vi "Read prelaunchSettings.vi"(8 "error in (no error)":errorcluster, 11 "ZM-ROOT-root in":refnum<class "ZM-ROOT-root.lvclass">) -> (0 "error out":errorcluster, 2 "ZM-ROOT-PRELAUNCH_SETTINGS":T1, 3 "ZM-ROOT-root out":refnum<class "ZM-ROOT-root.lvclass">)   [LabVIEW 2020, in "ZM-ROOT-root.lvlib" / "ZM-ROOT-root.lvclass"]
doc: "Reads one field of this class's private data. Generated by lvai_create_accessors from the class private data control."
uses:
  ZM-ROOT-root.lvclass
  ZM-ROOT-root.lvclass/ZM-ROOT-root.ctl
  ZM-ROOT-PRELAUNCH_SETTINGS.ctl
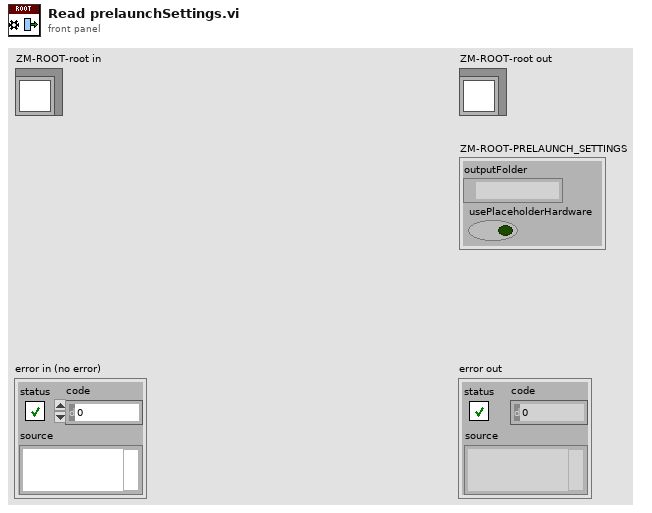
[diagram p1: front panel]
types:
  T1 = typedef "ZM-ROOT-root.lvlib/ZM-ROOT-root.lvclass/ZM-ROOT-PRELAUNCH_SETTINGS.ctl" = cluster{"outputFolder":path, "usePlaceholderHardware":bool}
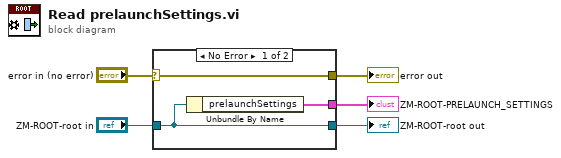
[diagram p0: block diagram]
diagram:
  n1 = case shown="No Error" "error in (no error)" {
    selector: "error in (no error)" -> [w8 w9]
    tunnel: [w8 w9] -> w4
    tunnel: [w7 w10] -> w2
    tunnel: "ZM-ROOT-root in" -> [w7 w10]
    tunnel: [w6 _] -> w1
    frame No Error {
      n2 = Unbundle By Name(w7) -> ("prelaunchSettings"=w6:T1)
    }
    frame Error {
    }
  }
  "error out" <- w4
  "ZM-ROOT-root out" <- w2
  "ZM-ROOT-PRELAUNCH_SETTINGS" <- w1
